vi "TblNameParam (SubVI).vi"(8 "error in (no error)":errorcluster) -> (0 "error out":errorcluster, 2 "Tbl1NameParam":string[](array[string]), 3 "Tbl0NameParam":string[](array[string]))   [LabVIEW 2017]
uses:
  Global_SNK3_HF.vi
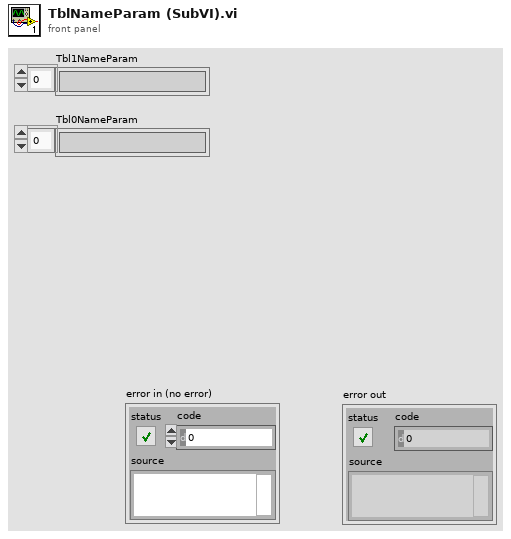
[diagram p1: front panel]
types:
  T1 = typedef "LV_Unicorn.lvlib/unicorn_Param.ctl" = cluster{"conParam":T2, "Param":T3}
  T2 = typedef "LV_Unicorn.lvlib/unicorn_conn.ctl" = cluster{"ReadIntParam":bool, "ReadDescrParam":bool, "ReadFloatParam":bool, "debug":bool, "ReadJSON":bool, "IP_address":string, "N_attempts":i32, "type_con":enum16{"Serial", "TCP"}, "MB_address":i32, "VISA":refnum<visa-resource-name>, "connection ID":refnum<k5>, "nameDevices":string, "timeout":i32, "port":u16, "type_version":string, "baud_rate":u32, "VersionControl":bool, "TCP_conn":bool, "WindowSize":i32}
  T3 = typedef "LV_Unicorn.lvlib/unicorn_JSON.ctl" = cluster{"NumParam":cluster{"NTelem":i32, "NInt":i32, "NFloat":i32, "NTable":i32}, "ParamInt":T4, "Telemetry":T5, "Table":T6, "ParamFloat":T7}
  T4 = typedef "LV_Unicorn.lvlib/unicorn_ParamInt.ctl" = cluster{"ID":string, "Num":i32, "Name":string, "Type":string, "Enum":string, "Desc":string, "Unit":string, "Access":string, "FormatStr":string, "Min":i32, "Max":i32}[]
  T5 = typedef "LV_Unicorn.lvlib/unicorn_Telemetry.ctl" = cluster{"ID":string, "Num":i32, "Name":string, "Desc":string, "Unit":string, "FormatStr":string, "Min":i32, "Max":i32}[]
  T6 = typedef "LV_Unicorn.lvlib/unicorn_Table.ctl" = cluster{"Num":i32, "Access":string, "ColumnCount":i32, "NeedParamPrepare":bool, "Columns":cluster{"Column":i32, "Desc":string, "Name":string}[], "DataType":string, "FormatStr":string, "ID":string, "Name":string, "RowCount":i32, "Rows":cluster{"Desc":string, "ID":string, "Max":i32, "Min":i32, "Name":string, "Row":i32, "Unit":string}[], "Type":string}[]
  T7 = typedef "LV_Unicorn.lvlib/unicorn_ParamFloat.ctl" = cluster{"ID":string, "Num":i32, "Name":string, "Type":string, "Enum":string, "Desc":string, "Unit":string, "Access":string, "FormatStr":string, "Min":sgl, "Max":sgl}[]
  T8 = cluster{"Num":i32, "Access":string, "ColumnCount":i32, "NeedParamPrepare":bool, "Columns":cluster{"Column":i32, "Desc":string, "Name":string}[], "DataType":string, "FormatStr":string, "ID":string, "Name":string, "RowCount":i32, "Rows":cluster{"Desc":string, "ID":string, "Max":i32, "Min":i32, "Name":string, "Row":i32, "Unit":string}[], "Type":string}
  T9 = cluster{"Desc":string, "ID":string, "Max":i32, "Min":i32, "Name":string, "Row":i32, "Unit":string}[]
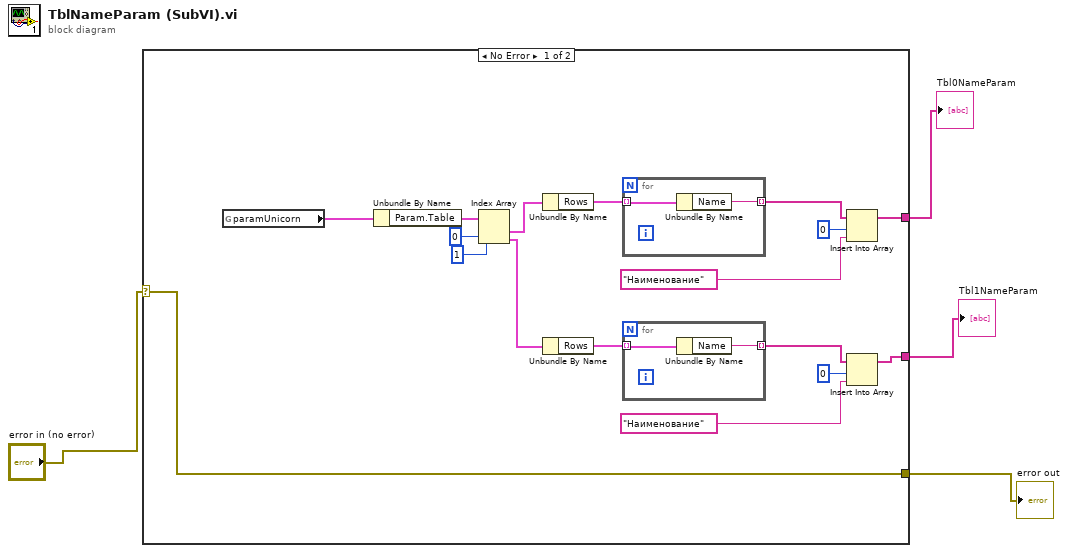
[diagram p0: block diagram]
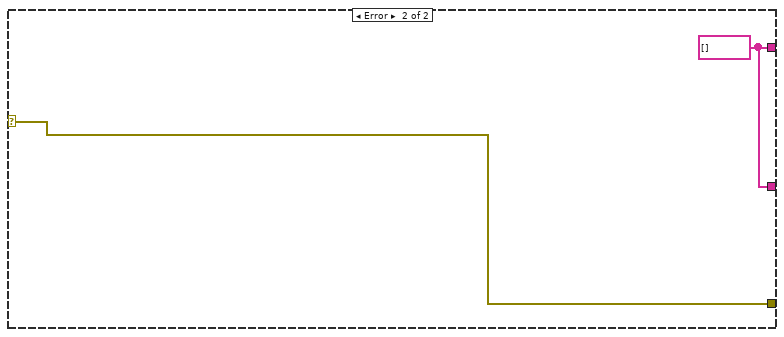
[diagram p2: hidden frame]
diagram:
  n1 = case shown="No Error" "error in (no error)" {
    selector: "error in (no error)" -> [w5 w27]
    tunnel: [w19 w26] -> w4
    tunnel: [w13 w26] -> w3
    tunnel: [w5 w27] -> w1
    frame No Error {
      n2 = global read "Global_SNK3_HF.vi" "paramUnicorn"() -> (w6:T1)
      n3 = Unbundle By Name(w6) -> ("Param.Table"=w8:T6)
      n4 = Index Array(array=w8, index #1=0 ("index"), index #2=1 ("index")) -> (element #1=w9:T8, element #2=w18:T8)
      n5 = Unbundle By Name(w9) -> ("Rows"=w10:T9)
      n6 = Unbundle By Name(w18) -> ("Rows"=w16:T9)
      n7 = for {
        tunnel: w10 -> [w25] mode=indexing
        tunnel: [w24] -> w12 mode=indexing
        n8 = Unbundle By Name(w25) -> ("Name"=w24:string)
      }
      n9 = for {
        tunnel: w16 -> [w23] mode=indexing
        tunnel: [w22] -> w14 mode=indexing
        n10 = Unbundle By Name(w23) -> ("Name"=w22:string)
      }
      n11 = Insert Into Array(array=w12, index=0, new element="Наименование") -> (w13:string[])
      n12 = Insert Into Array(array=w14, index=0, new element="Наименование") -> (w19:string[])
    }
    frame Error {
      w26 = string[] []
    }
  }
  "Tbl1NameParam" <- w4
  "Tbl0NameParam" <- w3
  "error out" <- w1
